vi "SA save Fundamental Screenshot.vi"(8 "error in (no error)":errorcluster caption="에러 입력(에러 없음)", 11 "Instrument Manager 입력":refnum<class "Instrument Manager.lvclass">) -> (0 "error out":errorcluster caption="에러 출력", 3 "Instrument Manager 출력":refnum<class "Instrument Manager.lvclass">)   [LabVIEW 2023, in "Instrument Manager.lvclass"]
uses:
  Instrument Manager.lvclass
  Instrument Manager.lvclass/Instrument Manager.ctl
  Module/Spectrum Analyzer/Interface_Spectrum/Interface_Spectrum.lvclass
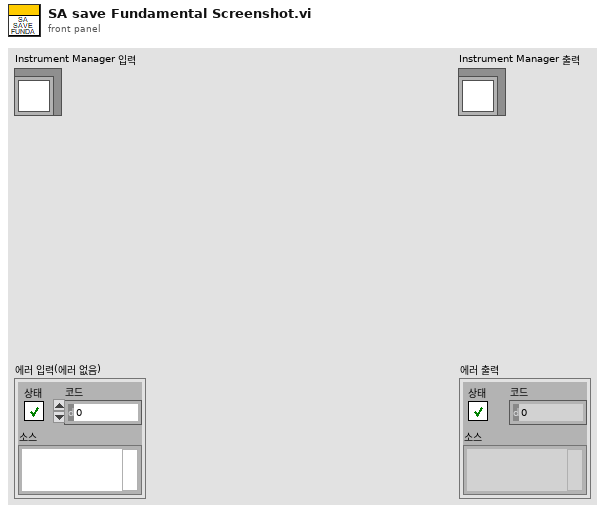
[diagram p1: front panel]
types:
  T1 = cluster{"Anritsu Call Box":refnum<class "Anritsu Call Box.lvclass">, "Spectrum Analyzer":refnum<class "Interface_Spectrum.lvclass">, "RF Switch Box":refnum<class "RF Filter Box.lvclass">, "Turn Table":refnum<class "Interface - Turn Table.lvclass">, "Mast":refnum<class "Interface - Mast.lvclass">, "3D Controller":refnum<class "Interface_3D Controller.lvclass">}
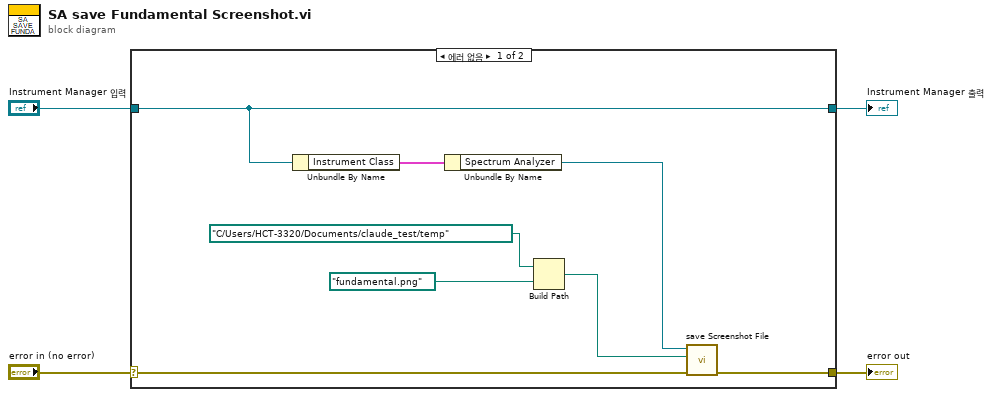
[diagram p0: block diagram]
diagram:
  n1 = case shown="에러 없음" "error in (no error)" {
    selector: "error in (no error)" -> [w7 w14]
    tunnel: [w6 w14] -> w3
    tunnel: [w5 w13] -> w1
    tunnel: "Instrument Manager 입력" -> [w5 w13]
    frame No Error {
      n2 = Unbundle By Name(w5) -> ("Instrument Class"=w11:T1)
      n3 = Unbundle By Name(w11) -> ("Spectrum Analyzer"=w12:refnum<class "Interface_Spectrum.lvclass">)
      n4 = Build Path(base path=path "C:/Users/HCT-3320/Documents/claude_test/temp" ("File Path"), name or relative path=path "fundamental.png" ("이름 또는 상대 경로")) -> (appended path=w10:path)
      n5 = call-dynamic "save Screenshot File.vi"("error in (no error)"=w7, "File Path"=w10, "Interface_Spectrum in"=w12) -> ("error out"=w6:errorcluster)  [unwired: 7 in, 1 out]
    }
    frame Error {
    }
  }
  "error out" <- w3
  "Instrument Manager 출력" <- w1
